vi "Launcher.vi"   [LabVIEW 2024]
uses:
  Viewmodel/Viewmodel.lvclass
  View/View.lvclass
panel:
  # "LAUNCHER"
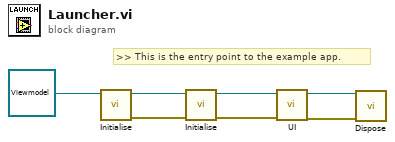
[diagram p0: block diagram]
diagram:
  # ">> This is the entry point to the example app."
  n1 = call-dynamic "Initialise.vi"("ChangeNotifier in"=refnum<class "Viewmodel.lvclass"> refnum ("Viewmodel.lvclass")) -> ("error out"=w1:errorcluster, "ChangeNotifier out"=w2:refnum<class "Viewmodel.lvclass">)  [unwired: 9 in]
  n2 = call "Initialise.vi"("error in (no error)"=w1, "Viewmodel"=w2) -> ("error out"=w6:errorcluster, "View out"=w7:refnum<class "View.lvclass">)  [unwired: 8 in]
  n3 = call "UI.vi"("error in (no error)"=w6, "View in"=w7) -> ("error out"=w4:errorcluster, "View out"=w5:refnum<class "View.lvclass">)  [unwired: 8 in]
  n4 = call "Dispose.vi"("error in (no error)"=w4, "View in"=w5) -> ()  [unwired: 8 in, 2 out]
